vi "usbpt104GetValue.vi"(7 "Channel":i32, 8 "error in (no error)":errorcluster, 11 "handle in":i16) -> (0 "error out":errorcluster, 2 "Channel Data":T1, 3 "handle out":i16)   [LabVIEW 2010]
doc: "Calls UsbPt104GetValue for single channel, returns single value."
uses:
  UsbPT104.dll
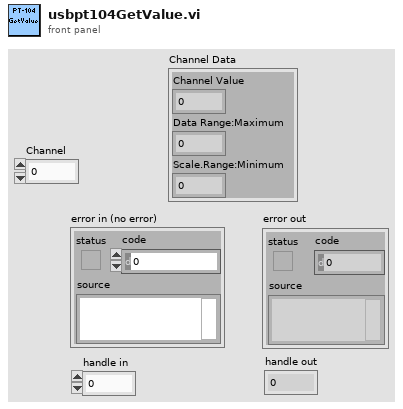
[diagram p1: front panel]
types:
  T1 = cluster{"Channel Value":dbl, "Data Range:Maximum":dbl, "Scale.Range:Minimum":dbl}
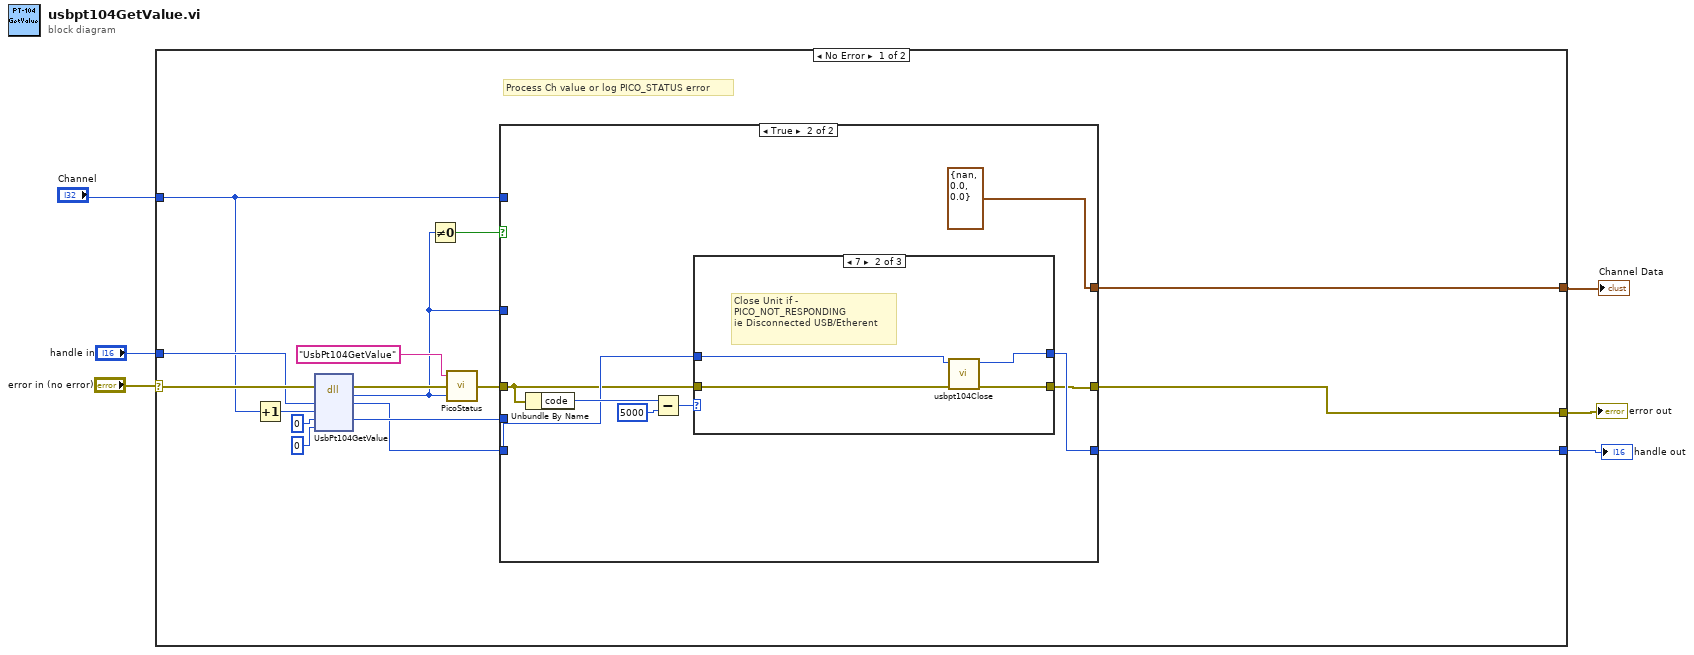
[diagram p0: block diagram]
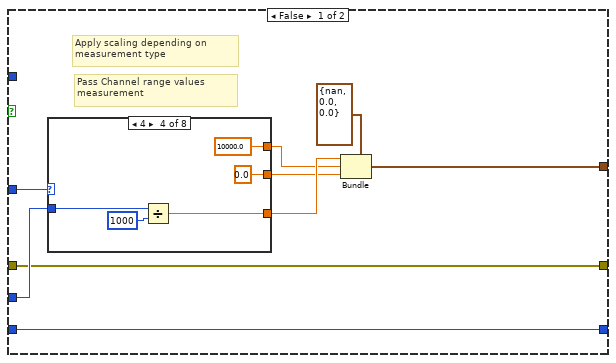
[diagram p2: hidden frame]
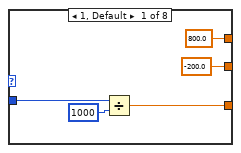
[diagram p3: hidden frame]
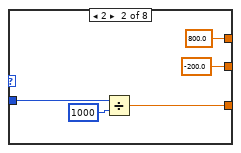
[diagram p4: hidden frame]
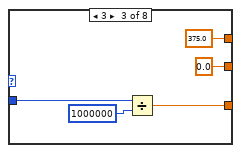
[diagram p5: hidden frame]
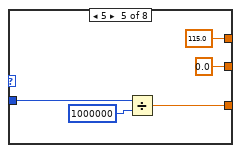
[diagram p6: hidden frame]
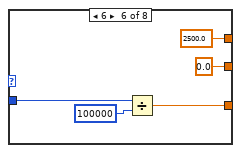
[diagram p7: hidden frame]
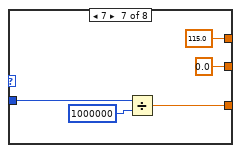
[diagram p8: hidden frame]
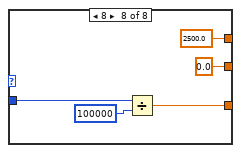
[diagram p9: hidden frame]
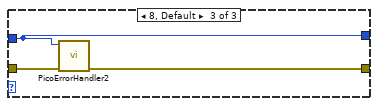
[diagram p11: hidden frame]
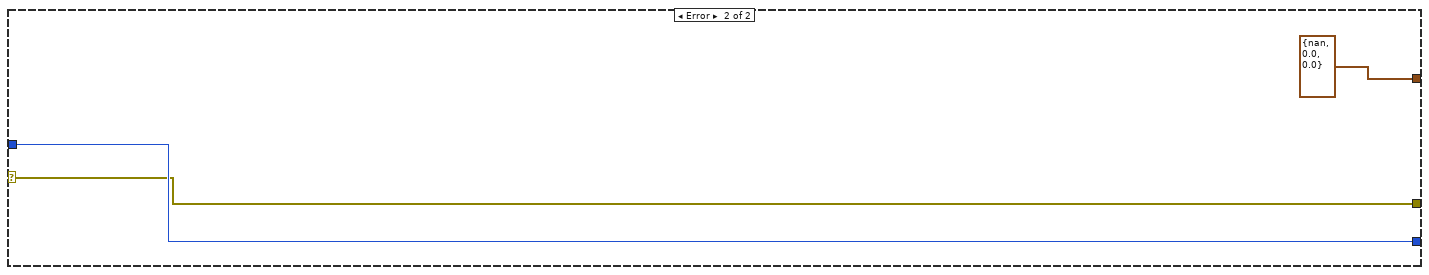
[diagram p12: hidden frame]
diagram:
  n1 = case shown="No Error" "error in (no error)" {
    selector: "error in (no error)" -> [w13 w90]
    tunnel: "handle in" -> [w12 w91]
    tunnel: [w10 w91] -> w6
    tunnel: [w11 w90] -> w5
    tunnel: "Channel" -> [w9 _]
    tunnel: [w7 T1 {"Channel Value"=nan, "Data Range:Maximum"=0.0, "Scale.Range:Minimum"=0.0} ("cluster")] -> w1
    frame No Error {
      # "Process Ch value or log PICO_STATUS error"
      n2 = Increment(x=w9) -> (x+1=w15:i32)
      n3 = dll-call lib="UsbPT104.dll" fn="UsbPt104GetValue"(error in=w13, "handle"=w12, "channel"=w15, "value"=0, "filtered"=i16 0) -> (error out=w20:errorcluster, "PICO_STATUS"=w8:u32, "handle"=w14:i16, "value"=w18:i32)  [unwired: 4 in, 1 out]
      n4 = Not Equal To 0?(x=w8) -> (x != 0?=w19:bool)
      n5 = call "PicoStatus.vi"("PICO STATUS"=w8, "error in"=w20, "source"="UsbPt104GetValue") -> ("error out"=w17:errorcluster)
      n6 = case shown="True" w19 {
        tunnel: w17 -> [w29 w75]
        tunnel: w18 -> [w31 _]
        tunnel: w9 -> [_ _]
        tunnel: w14 -> [w30 w76]
        tunnel: [w30 w74] -> w10
        tunnel: [w29 w73] -> w11
        tunnel: w8 -> [w28 _]
        tunnel: [w23 T1 {"Channel Value"=nan, "Data Range:Maximum"=0.0, "Scale.Range:Minimum"=0.0} ("cluster")] -> w7
        frame False {
          # "Pass Channel range values measurement"
          # "Apply scaling depending on \nmeasurement type"
          n7 = case shown="4" w28 {
            tunnel: w31 -> [w35 w40 w45 w50 w55 w60 w65 w70]
            tunnel: [w34 w39 w44 w49 w54 w59 w64 w69] -> w27
            tunnel: [800.0 ("Data Range:Maximum") 800.0 ("Data Range:Maximum") 375.0 ("Data Range:Maximum") 10000.0 ("Data Range:Maximum") 115.0 ("Data Range:Maximum") 2500.0 ("Data Range:Maximum") 115.0 ("Data Range:Maximum") 2500.0 ("Data Range:Maximum")] -> w26
            tunnel: [-200.0 ("Scale.Range:Minimum") -200.0 ("Scale.Range:Minimum") 0.0 ("Scale.Range:Minimum") 0.0 ("Scale.Range:Minimum") 0.0 ("Scale.Range:Minimum") 0.0 ("Scale.Range:Minimum") 0.0 ("Scale.Range:Minimum") 0.0 ("Scale.Range:Minimum")] -> w25
            frame 1, Default {
              n8 = Divide(x=w35, y=1000) -> (x/y=w34:dbl)
            }
            frame 2 {
              n9 = Divide(x=w40, y=1000) -> (x/y=w39:dbl)
            }
            frame 3 {
              n10 = Divide(x=w45, y=1000000) -> (x/y=w44:dbl)
            }
            frame 4 {
              n11 = Divide(x=w50, y=1000) -> (x/y=w49:dbl)
            }
            frame 5 {
              n12 = Divide(x=w55, y=1000000) -> (x/y=w54:dbl)
            }
            frame 6 {
              n13 = Divide(x=w60, y=100000) -> (x/y=w59:dbl)
            }
            frame 7 {
              n14 = Divide(x=w65, y=1000000) -> (x/y=w64:dbl)
            }
            frame 8 {
              n15 = Divide(x=w70, y=100000) -> (x/y=w69:dbl)
            }
          }
          n16 = Bundle(cluster=T1 {"Channel Value"=nan, "Data Range:Maximum"=0.0, "Scale.Range:Minimum"=0.0}, "Channel Value"=w27, "Data Range:Maximum"=w26, "Scale.Range:Minimum"=w25) -> (w23:T1)
        }
        frame True {
          n17 = Unbundle By Name(w75) -> ("code"=w79:i32)
          n18 = Subtract(x=w79, y=5000) -> (x-y=w77:i32)
          n19 = case shown="7" w77 {
            tunnel: w76 -> [w81 w85 w87]
            tunnel: w75 -> [w80 w84 w88]
            tunnel: [w81 w83 w87] -> w74
            tunnel: [w80 w82 w86] -> w73
            frame 37 {
              # "Data is unavailable because a run\nhas not been completed.\nPICO_NO_SAMPLES_AVAILABLE \n0x00000025UL"
            }
            frame 7 {
              # "Close Unit if -\nPICO_NOT_RESPONDING\nie Disconnected USB/Etherent"
              n20 = call "usbpt104Close.vi"("error in (no error)"=w84, "handle in"=w85) -> ("error out"=w82:errorcluster, "handle out"=w83:i16)  [unwired: 8 in]
            }
            frame 8, Default {
              n21 = call "PicoErrorHandler2.vi"("error in (no error)"=w88, "handle In"=w87) -> ("error out"=w86:errorcluster)  [unwired: 9 in]
            }
          }
        }
      }
    }
    frame Error {
    }
  }
  "error out" <- w5
  "handle out" <- w6
  "Channel Data" <- w1
